vi "Intake Teleop Handler.vi"() -> ()   [LabVIEW 2025]
uses:
  <vilib>/Rock Robotics/WPI/Joystick/XBox Axes Indexer.ctl
  Shooter/Implementation/Shooter Modes.ctl
  14dd900b-f513-4e9f-930a-5a9299410501.vi
  2fbf93c8-80ea-446d-afa8-816ad16bbded.vi
  eea64580-3f51-4283-881f-b83a8d73652c.vi
  58505169-8ced-43df-a5a8-20a0a13db2fe.vi
  fbf58d8b-d6f4-4204-94d0-91bce9191d94.vi
  e08305e5-bdc7-4cb8-b859-a13f5bfcab12.vi
  693ed9fc-a9b3-4ade-88be-bc30baa6b2f9.vi
  6deef821-4a13-4ad9-a755-ca3546996214.vi
  83387108-919a-4e0e-b432-a0e502da9ea5.vi
  <vilib>/Rock Robotics/WPI/Utilities/WPI_GetSetVariantRefNum.vi
  Framework/Robot Global Data.vi
panel:
  in  "Transfering Intake Speed":dbl=1750.0
  in  "Stowed V Hopper Pos":dbl
  in  "Extended V Hopper Pos":dbl=10.8
  in  "Extended Intake Pos":dbl=24.0
  in  "Intake Speed":dbl=4000.0
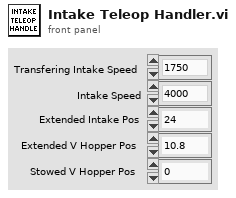
[diagram p1: front panel]
types:
  T1 = typedef "XBox Axes Indexer.ctl" = enum16{"Left X", "Left Y", "Left Trigger", "Right Trigger", "Right X", "Right Y"}
  T2 = typedef "Shooter Modes.ctl" = enum16{"C to A Close", "C to A Far", "A to A", "Tower", "Interp", "Idle"}
  T3 = typedef "WPI_JoystickDevRef.ctl" = cluster{"Device":T4}
  T4 = typedef "WPI_JoystickDeviceEnum.ctl" = enum16{"USB 0", "USB 1", "USB 2", "USB 3", "USB 4", "USB 5"}
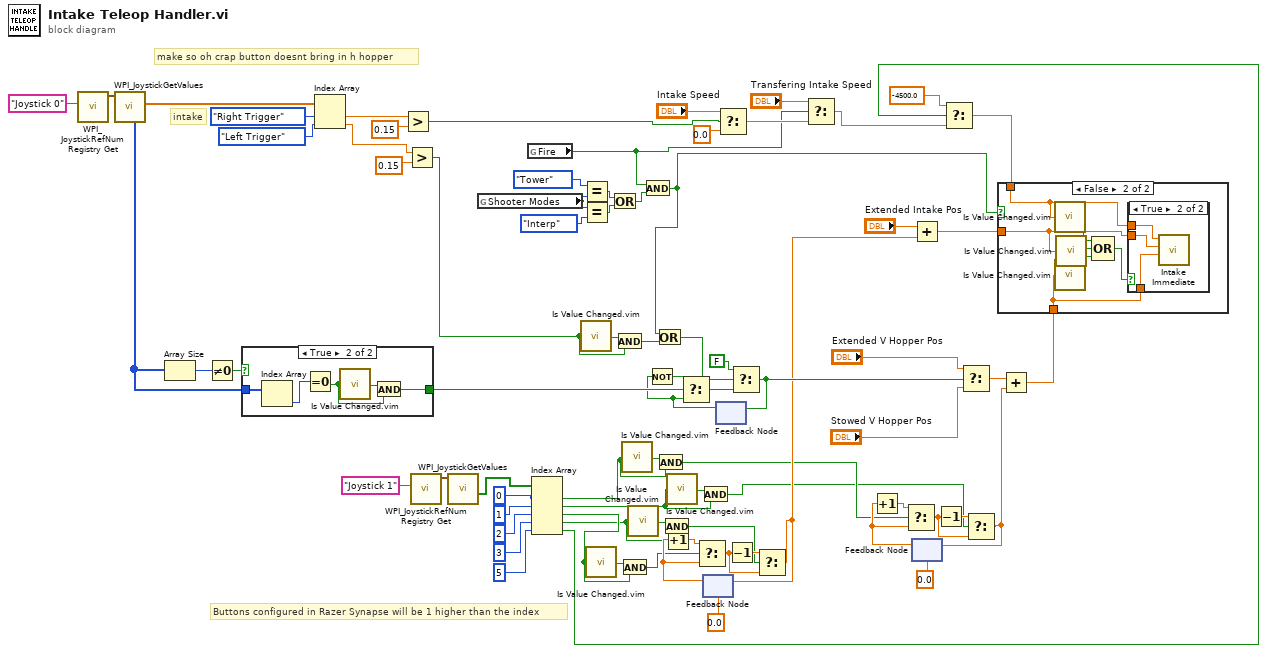
[diagram p0: block diagram]
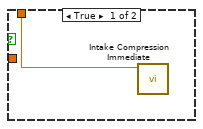
[diagram p2: hidden frame]
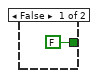
[diagram p4: hidden frame]
diagram:
  # "Buttons configured in Razer Synapse will be 1 higher than the index"
  # "make so oh crap button doesnt bring in h hopper"
  # "intake"
  n1 = call <vilib>:"WPI_JoystickRefNum Registry Get.vi"("refnum name"="Joystick 0") -> ("JoystickDevRef"=w76:T3)  [unwired: 1 in, 9 out]
  n2 = call <vilib>:"WPI_JoystickGetValues.vi"("JoystickDevRef"=w76) -> ("Axes"=w75:dbl[], "POVs"=w67:i16[])  [unwired: 6 in, 3 out]
  n3 = Array Size(array=w67) -> (size(s)=w69:i32)
  n4 = Not Equal To 0?(x=w69) -> (x != 0?=w68:bool)
  n5 = case shown="True" w68 {
    tunnel: w67 -> [_ w83]
    tunnel: [FALSE w80] -> w57
    frame False {
    }
    frame True {
      n6 = Index Array(array=w83) -> (element=w79:i16)  [unwired: 1 in]
      n7 = Equal To 0?(x=w79) -> (x = 0?=w82:bool)
      n8 = call "Is Value Changed.vim"("value"=w82) -> ("changed or first call?"=w81:bool)
      n9 = And(x=w81, y=w82) -> (x .and. y?=w80:bool)
    }
  }
  n10 = Index Array(array=w75, index #1=XBox_Axes_Indexer."Right Trigger" ("XBox Axes"), index #2=XBox_Axes_Indexer."Left Trigger" ("XBox Axes")) -> (element #1=w74:dbl, element #2=w16:dbl)
  n11 = Greater?(x=w74, y=0.15) -> (0:w4:bool)
  n12 = Greater?(x=w16, y=0.15) -> (0:w15:bool)
  n13 = call <vilib>:"WPI_JoystickRefNum Registry Get.vi"("refnum name"="Joystick 1") -> ("JoystickDevRef"=w53:T3)  [unwired: 1 in, 9 out]
  n14 = call <vilib>:"WPI_JoystickGetValues.vi"("JoystickDevRef"=w53) -> ("Buttons"=w46:bool[])  [unwired: 6 in, 4 out]
  n15 = global read "Robot Global Data.vi" "Shooter Modes"() -> (w66:T2)
  n16 = global read "Robot Global Data.vi" "Fire"() -> (w3:bool)
  n17 = Index Array(array=w46, index #1=0 ("index"), index #2=1 ("index"), index #3=2 ("index"), index #4=3 ("index"), index #5=5 ("index")) -> (element #1=w30:bool, element #2=w26:bool, element #3=w24:bool, element #4=w21:bool, element #5=w9:bool)
  n18 = call "Is Value Changed.vim"("value"=w15) -> ("changed or first call?"=w18:bool)
  n19 = Equal?(x=Shooter_Modes."Tower", y=w66) -> (x = y?=w63:bool)
  n20 = Equal?(x=w66, y=Shooter_Modes."Interp") -> (x = y?=w62:bool)
  n21 = call "Is Value Changed.vim"("value"=w24) -> ("changed or first call?"=w25:bool)
  n22 = Or(x=w63, y=w62) -> (x .or. y?=w61:bool)
  n23 = And(x=w18, y=w15) -> (x .and. y?=w14:bool)
  n24 = And(x=w25, y=w24) -> (x .and. y?=w23:bool)
  n25 = call "Is Value Changed.vim"("value"=w30) -> ("changed or first call?"=w31:bool)
  n26 = call "Is Value Changed.vim"("value"=w21) -> ("changed or first call?"=w22:bool)
  n27 = And(x=w3, y=w61) -> (x .and. y?=w5:bool)
  n28 = Or(x=w5, y=w14) -> (x .or. y?=w19:bool)
  n29 = And(x=w31, y=w30) -> (x .and. y?=w29:bool)
  n30 = And(x=w22, y=w21) -> (x .and. y?=w20:bool)
  n31 = call "Is Value Changed.vim"("value"=w26) -> ("changed or first call?"=w28:bool)
  n32 = And(x=w28, y=w26) -> (x .and. y?=w27:bool)
  n33 = feedback #1(0.0) -> (w37:dbl)
  n34 = Increment(x=w37) -> (x+1=w40:dbl)
  n35 = Select(t=w40, s=w23, f=w37) -> (s? t:f=w38:dbl)
  n36 = feedback #2() -> (w56:bool)  [unwired: 1 in]
  n37 = Not(x=w56) -> (.not. x?=w58:bool)
  n38 = Select(t=w58, s=w57, f=w56) -> (s? t:f=w60:bool)
  n39 = Select(t="Intake Speed", s=w4, f=0.0) -> (s? t:f=w7:dbl)
  n40 = Decrement(x=w38) -> (x-1=w39:dbl)
  n41 = Select(t=FALSE, s=w19, f=w60) -> (s? t:f=w55:bool)
  n42 = feedback-in #2(w55) -> ()
  n43 = Select(t=w39, s=w20, f=w38) -> (s? t:f=w34:dbl)
  n44 = feedback-in #1(w34) -> ()
  n45 = Select(t="Transfering Intake Speed", s=w3, f=w7) -> (s? t:f=w6:dbl)
  n46 = Add(x="Extended Intake Pos", y=w34) -> (x+y=w35:dbl)
  n47 = feedback #3(0.0) -> (w42:dbl)
  n48 = Increment(x=w42) -> (x+1=w45:dbl)
  n49 = Select(t=w45, s=w29, f=w42) -> (s? t:f=w43:dbl)
  n50 = Decrement(x=w43) -> (x-1=w44:dbl)
  n51 = Select(t=-4500.0, s=w9, f=w6) -> (s? t:f=w12:dbl)
  n52 = Select(t="Extended V Hopper Pos", s=w55, f="Stowed V Hopper Pos") -> (s? t:f=w1:dbl)
  n53 = Select(t=w44, s=w27, f=w43) -> (s? t:f=w41:dbl)
  n54 = feedback-in #3(w41) -> ()
  n55 = Add(x=w1, y=w41) -> (x+y=w52:dbl)
  n56 = case shown="False" w5 {
    tunnel: w12 -> [w84 w87]
    tunnel: w52 -> [_ w86]
    tunnel: w35 -> [_ w85]
    frame True {
      n57 = call "Intake Compression Immediate.vi"("Intake Roller Speed"=w84) -> ()  [unwired: 10 in, 1 out]
    }
    frame False {
      n58 = call "Is Value Changed.vim"("value"=w87) -> ("changed or first call?"=w91:bool)
      n59 = call "Is Value Changed.vim"("value"=w86) -> ("changed or first call?"=w89:bool)
      n60 = call "Is Value Changed.vim"("value"=w85) -> ("changed or first call?"=w90:bool)
      n61 = Compound Arithmetic op=OR(w91, w90, w89) -> (w88:bool)
      n62 = case shown="True" w88 {
        tunnel: w87 -> [_ w94]
        tunnel: w85 -> [_ w93]
        tunnel: w86 -> [_ w92]
        frame False {
        }
        frame True {
          n63 = call "Intake Immediate.vi"("V Hopper Pos"=w92, "Intake Pivot Pos"=w93, "Intake Roller Speed"=w94) -> ()  [unwired: 8 in, 1 out]
        }
      }
    }
  }
